vi "xnet_canopen_write_batch.vi"(8 "error in (no error)":errorcluster, 10 "OD Batch in":refnum<class "OD Batch.lvclass">, 11 "xnet_co_handle_in":u64) -> (0 "error out":errorcluster, 2 "OD Batch":refnum<class "OD Batch.lvclass">, 3 "xnet_co_handle":u64)   [LabVIEW 2023, in "xnet_canopen.lvlib"]
uses:
  OD Batch/OD Batch.lvclass
  OD Batch/OD Batch.lvclass/OD Batch.ctl
  <vilib>/Utility/error.llb/Error Cluster From Error Code.vi
  xnet_canopen.lvlib
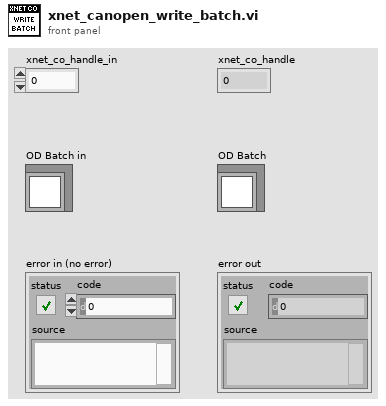
[diagram p1: front panel]
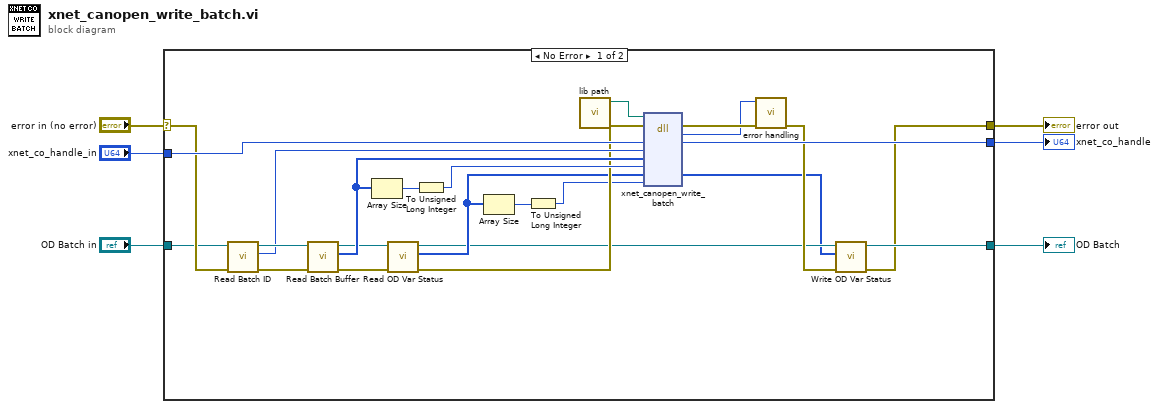
[diagram p0: block diagram]
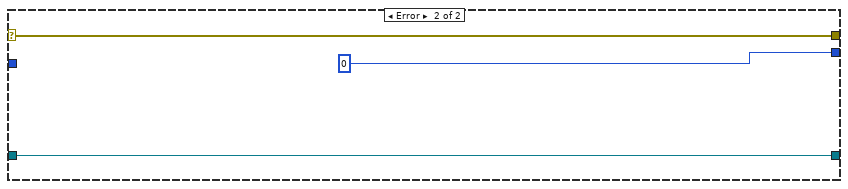
[diagram p2: hidden frame]
diagram:
  n1 = case shown="No Error" "error in (no error)" {
    selector: "error in (no error)" -> [w25 w33]
    tunnel: [w7 w33] -> w5
    tunnel: [w27 u64 0 ("phandle")] -> w4
    tunnel: "xnet_co_handle_in" -> [w26 _]
    tunnel: "OD Batch in" -> [w23 w31]
    tunnel: [w8 w31] -> w1
    frame No Error {
      n2 = call "Read Batch ID.vi"("error in (no error)"=w25, "OD Batch in"=w23) -> ("error out"=w24:errorcluster, "Batch ID"=w21:u32, "OD Batch out"=w22:refnum<class "OD Batch.lvclass">)  [unwired: 7 in]
      n3 = call "Read Batch Buffer.vi"("error in (no error)"=w24, "OD Batch in"=w22) -> ("error out"=w20:errorcluster, "Batch Buffer"=w19:u8[], "OD Batch out"=w15:refnum<class "OD Batch.lvclass">)  [unwired: 7 in]
      n4 = Array Size(array=w19) -> (size(s)=w18:i32)
      n5 = call "Read OD Var Status.vi"("error in (no error)"=w20, "OD Batch in"=w15) -> ("error out"=w16:errorcluster, "OD Var Status"=w14:i32[], "OD Batch out"=w10:refnum<class "OD Batch.lvclass">)  [unwired: 7 in]
      n6 = To Unsigned Long Integer(number=w18) -> (unsigned 32bit integer=w17:u32)
      n7 = Array Size(array=w14) -> (size(s)=w13:i32)
      n8 = To Unsigned Long Integer(number=w13) -> (unsigned 32bit integer=w12:u32)
      n9 = call "lib path.vi"() -> ("lib path"=w30:path)  [unwired: 11 in]
      n10 = dll-call lib="?" fn="xnet_canopen_write_batch"(path in=w30, error in=w16, "handle"=w26, "batch_id"=w21, "buffer"=w19, "bufsize"=w17, "entry_status"=w14, "entry_cnt"=w12) -> (error out=w29:errorcluster, "return type"=w28:i32, "handle"=w27:u64, "entry_status"=w9:i32[])  [unwired: 5 in, 1 out]
      n11 = call "error handling.vi"("error in (no error)"=w29, "return val"=w28) -> ("error out"=w11:errorcluster)  [unwired: 9 in]
      n12 = call "Write OD Var Status.vi"("error in (no error)"=w11, "OD Var Status"=w9, "OD Batch in"=w10) -> ("error out"=w7:errorcluster, "OD Batch out"=w8:refnum<class "OD Batch.lvclass">)  [unwired: 7 in]
    }
    frame Error {
    }
  }
  "error out" <- w5
  "xnet_co_handle" <- w4
  "OD Batch" <- w1
